vi "OwnMethod20261013_SetWireRule.vi"() -> ()   [LabVIEW 2024]
panel:
  out "error out":errorcluster caption="错误输出"
  in  "Rule":T1(ring)
  in  "TermIdx":u32
  in  "target_path":path
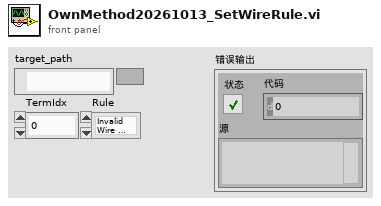
[diagram p1: front panel]
types:
  T1 = enum16{"Invalid Wire Rule", "Required", "Recommended", "Optional", "Dynamic Dispatch"}
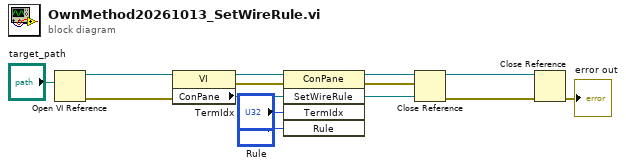
[diagram p0: block diagram]
diagram:
  n1 = Open VI Reference(vi path="target_path") -> (vi reference=w9:refnum<vi>, error out=w8:errorcluster)  [unwired: 5 in]
  n2 = property class="VI"(reference=w9, error in=w8) -> (error out=w6:errorcluster, "ConPane"=w7:refnum<vi>)  [unwired: 1 out]
  n3 = invoke class="ConPane" method="SetWireRule"(reference=w7, error in=w6, "TermIdx"="TermIdx", "Rule"="Rule") -> (error out=w3:errorcluster)  [unwired: 1 in, 4 out]
  n4 = Close Reference(reference=w7, error in (no error)=w3) -> (error out=w2:errorcluster)
  n5 = Close Reference(reference=w9, error in (no error)=w2) -> (error out=→"error out":errorcluster)
